vi "Is Running.vi"() -> (0 "is running?":bool)   [LabVIEW 2018, in "GLog.lvlib" / "Registry.lvlib"]
uses:
  Registry.lvlib
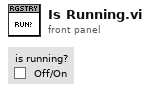
[diagram p1: front panel]
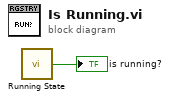
[diagram p0: block diagram]
diagram:
  n1 = call "Running State.vi"() -> ("value out"=→"is running?":bool)  [unwired: 2 in]
